vi "Save_Log.vi"(0 "日志文件路径":path, 1 "错误输入":errorcluster, 2 "日志记录行":string, 4 "打开或新建":T1(ring)=enum."open or create", 5 "写入位置（末尾）":enum16{"start", "end", "current"}(ring)=enum."end") -> (3 "错误输出":errorcluster)   [LabVIEW 2020]
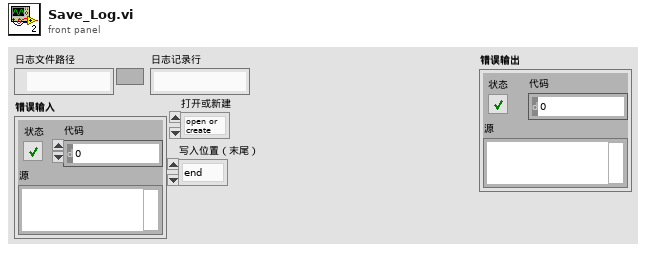
[diagram p1: front panel]
types:
  T1 = enum16{"open", "replace", "create", "open or create", "replace or create", "replace or create with confirmation"}
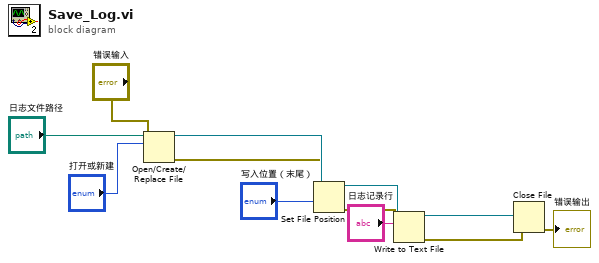
[diagram p0: block diagram]
diagram:
  n1 = Open/Create/Replace File(file path (use dialog)="日志文件路径", error in="错误输入", operation (0:open)="打开或新建") -> (refnum out=w6:refnum<file>, error out=w5:errorcluster)  [unwired: 3 in, 1 out]
  n2 = Set File Position(refnum=w6, from (0:start)="写入位置（末尾）", error in=w5) -> (refnum out=w4:refnum<file>, error out=w3:errorcluster)  [unwired: 1 in]
  n3 = Write to Text File(file (use dialog)=w4, text="日志记录行", error in=w3) -> (refnum out=w2:refnum<file>, error out=w1:errorcluster)  [unwired: 1 in, 1 out]
  n4 = Close File(refnum=w2, error in=w1) -> (error out=→"错误输出":errorcluster)  [unwired: 1 out]
